vi "Measure Harmonic.vi"(8 "error in (no error)":errorcluster caption="에러 입력(에러 없음)", 10 "Fundametal Freq":dbl, 11 "Instrument Manager 입력":refnum<class "Instrument Manager.lvclass">) -> (0 "error out":errorcluster caption="에러 출력", 1 "Frequency":dbl[](array[numeric]), 2 "Amplitude":dbl[](array[numeric]), 3 "Instrument Manager 출력":refnum<class "Instrument Manager.lvclass">)   [LabVIEW 2023, in "Instrument Manager.lvclass"]
uses:
  Instrument Manager.lvclass
  Instrument Manager.lvclass/Instrument Manager.ctl
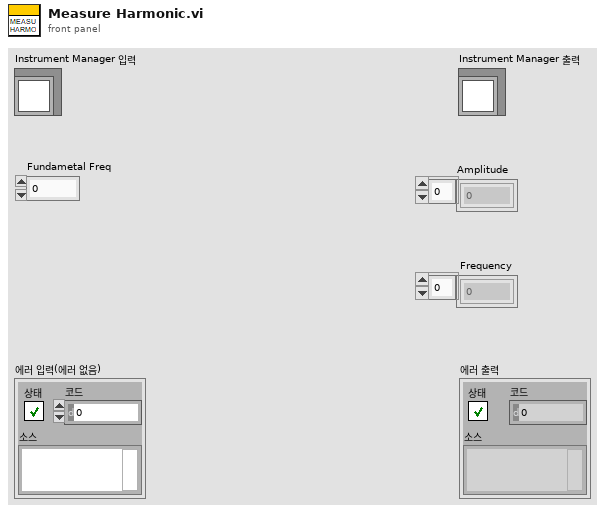
[diagram p1: front panel]
types:
  T1 = typedef "Spectrum Analyzer.lvlib/TYPE Trace Value Array.ctl" = cluster{"Frequency":dbl[], "Amplitude":dbl[]}
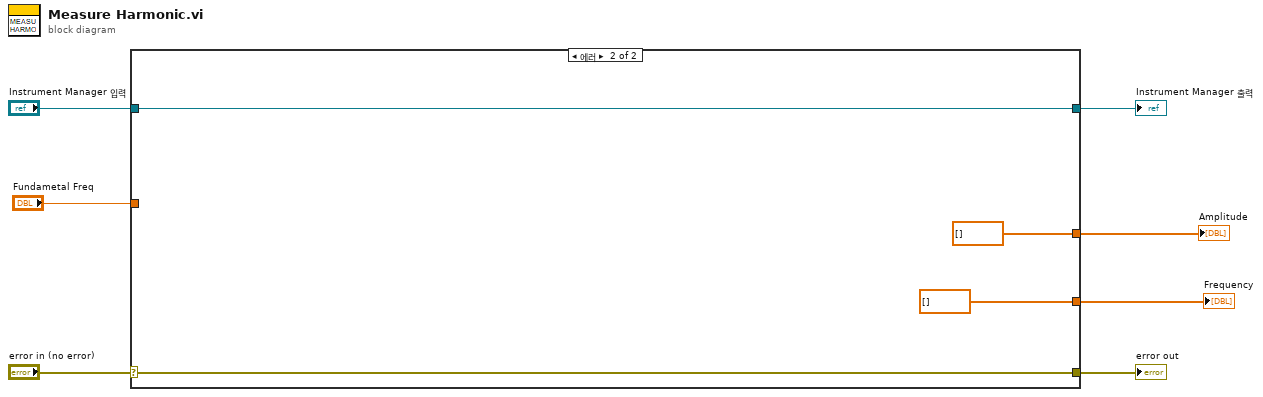
[diagram p0: block diagram]
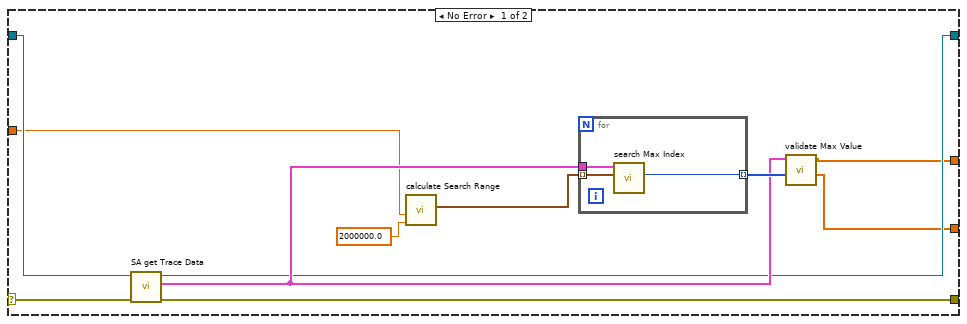
[diagram p2: hidden frame]
diagram:
  n1 = case shown="에러" "error in (no error)" {
    selector: "error in (no error)" -> [w14 w25]
    tunnel: [w11 w24] -> w5
    tunnel: "Instrument Manager 입력" -> [w12 w24]
    tunnel: [w13 w25] -> w4
    tunnel: "Fundametal Freq" -> [w10 _]
    tunnel: [w9 dbl[] [] ("Amplitude")] -> w2
    tunnel: [w8 dbl[] [] ("Frequency")] -> w1
    frame No Error {
      n2 = call "SA get Trace Data.vi"("error in (no error)"=w14, "Instrument Manager 입력"=w12) -> ("error out"=w13:errorcluster, "Trace Values"=w16:T1, "Instrument Manager 출력"=w11:refnum<class "Instrument Manager.lvclass">)  [unwired: 7 in]
      n3 = call "calculate Search Range.vi"("Search Width"=2000000.0, "Fundametal Freq"=w10) -> ("배열"=w17:cluster{"Start":dbl, "End":dbl}[])  [unwired: 9 in]
      n4 = for {
        tunnel: w17 -> [w21] mode=indexing
        tunnel: w16 -> [w19]
        tunnel: [w20] -> w18 mode=indexing
        n5 = call "search Max Index.vi"("Trace Values"=w19, "Search Range"=w21) -> ("Index"=w20:i32)  [unwired: 8 in]
      }
      n6 = call "validate Max Value.vi"("Max Index"=w18, "Trace Values"=w16) -> ("Frequency"=w8:dbl[], "Amplitude"=w9:dbl[])  [unwired: 7 in, 1 out]
    }
    frame Error {
    }
  }
  "error out" <- w4
  "Instrument Manager 출력" <- w5
  "Amplitude" <- w2
  "Frequency" <- w1
